vi "Dispose.vi"(8 "error in (no error)":errorcluster, 11 "Provider in":refnum<class "Provider.lvclass">) -> (0 "error out":errorcluster, 3 "Provider out":refnum<class "Provider.lvclass">)   [LabVIEW 2024, in "Provider.lvclass"]
uses:
  Provider.lvclass
  Provider.lvclass/Provider.ctl
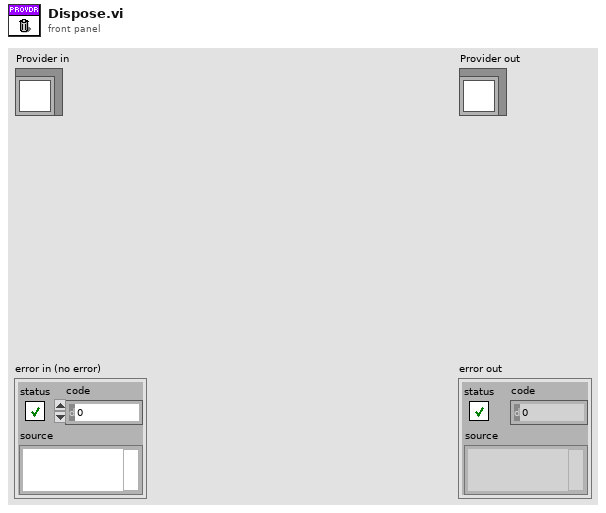
[diagram p1: front panel]
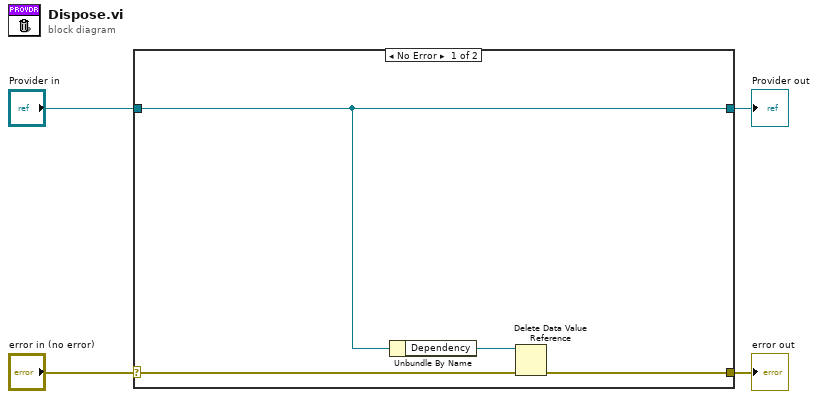
[diagram p0: block diagram]
diagram:
  n1 = case shown="No Error" "error in (no error)" {
    selector: "error in (no error)" -> [w8 w10]
    tunnel: [w7 w10] -> w3
    tunnel: [w6 w9] -> w1
    tunnel: "Provider in" -> [w6 w9]
    frame No Error {
      n2 = Unbundle By Name(w6) -> ("Dependency"=w5:refnum<data-value>)
      n3 = Delete Data Value Reference(data value reference=w5, error in=w8) -> (error out=w7:errorcluster)  [unwired: 1 out]
    }
    frame Error {
    }
  }
  "error out" <- w3
  "Provider out" <- w1
